vi "Clear.vi"(8 "error in (no error)":errorcluster, 11 "Execution UI In":refnum<class "Execution UI.lvclass">) -> (0 "error out":errorcluster)   [LabVIEW 2020, in "Execution UI.lvclass"]
uses:
  Execution UI.lvclass
  Result Model/Result Model.lvclass
  Framework/Configuration Manager/Configuration Manager.lvclass
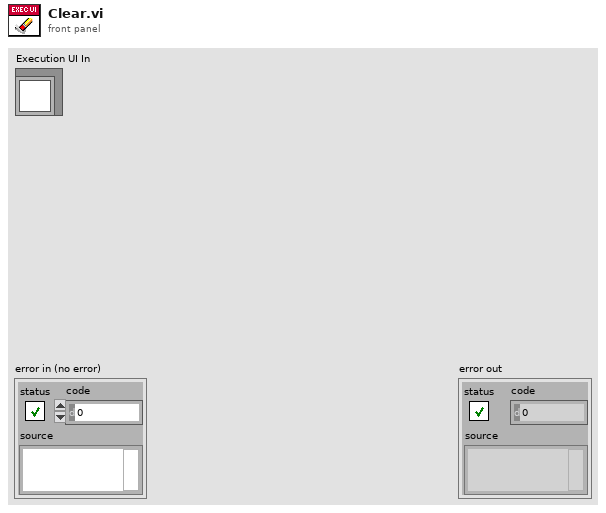
[diagram p1: front panel]
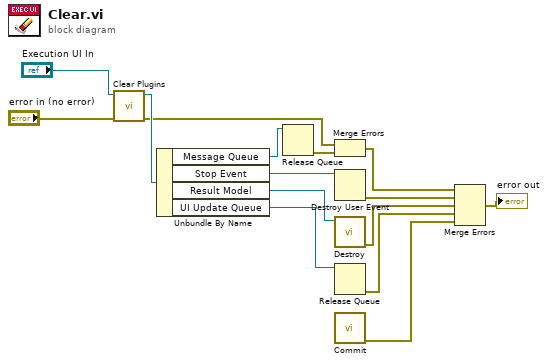
[diagram p0: block diagram]
diagram:
  n1 = call "Clear Plugins.vi"("error in (no error)"="error in (no error)", "Execution UI in"="Execution UI In") -> ("error out"=w5:errorcluster, "Execution UI out"=w6:refnum<class "Execution UI.lvclass">)  [unwired: 8 in]
  n2 = Unbundle By Name(w6) -> ("Message Queue"=w2:refnum<queue>, "Stop Event"=w13:refnum<user-event>, "Result Model"=w11:refnum<class "Result Model.lvclass">, "UI Update Queue"=w9:refnum<queue>)
  n3 = Release Queue(queue=w2) -> (error out=w3:errorcluster)  [unwired: 2 in, 2 out]
  n4 = Merge Errors(w5, w3) -> (w4:errorcluster)
  n5 = Destroy User Event(user event=w13) -> (error out=w12:errorcluster)  [unwired: 1 in]
  n6 = call "Destroy.vi"("Result Model in"=w11) -> ("error out"=w10:errorcluster)  [unwired: 10 in]
  n7 = Release Queue(queue=w9) -> (error out=w8:errorcluster)  [unwired: 2 in, 2 out]
  n8 = call "Commit.vi"() -> ("error out"=w1:errorcluster)  [unwired: 11 in]
  n9 = Merge Errors(w4, w12, w10, w8, w1) -> (→"error out":errorcluster)
